vi "Read Value Type Code.vi"(8 "error in (no error)":errorcluster, 11 "NT Scalar in":refnum<class "NT Scalar.lvclass">) -> (0 "error out":errorcluster, 2 "type code":T1, 3 "NT Scalar out":refnum<class "NT Scalar.lvclass">)   [LabVIEW 2020, in "PV Access.lvlib" / "PV Data.lvlib" / "NT Scalar.lvclass"]
uses:
  NT Scalar.lvclass
  NT Scalar.lvclass/NT Scalar.ctl
  1adc147a-9979-490a-b216-bcb4445dfe4b.vi
  Type Code.ctl
  PV Data.lvlib
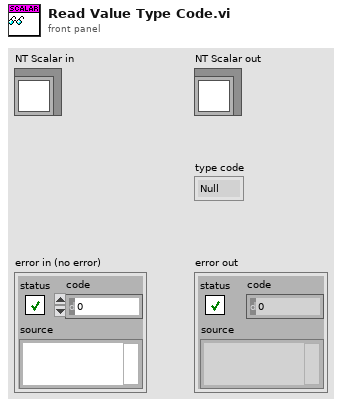
[diagram p1: front panel]
types:
  T1 = typedef "PV Access.lvlib/PV Data.lvlib/Type Code.ctl" = enum8{"Null", "Bool", "BoolA", "Int8", "Int8A", "Int16", "Int16A", "Int32", "Int32A", "Int64", "Int64A", "UInt8", "UInt8A", "UInt16", "UInt16A", "UInt32", "UInt32A", "UInt64", "UInt64A", "Float32", "Float32A", "Float64", "Float64A", "String", "StringA", "Struct", "StructA", "Union", "UnionA", "Any", "AnyA"}
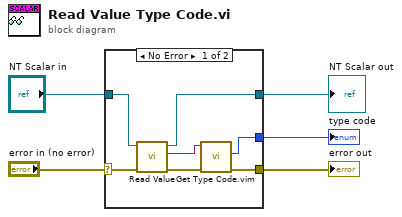
[diagram p0: block diagram]
diagram:
  n1 = case shown="No Error" "error in (no error)" {
    selector: "error in (no error)" -> [w10 w13]
    tunnel: [w7 w13] -> w4
    tunnel: [w11 w14] -> w2
    tunnel: "NT Scalar in" -> [w12 w14]
    tunnel: [w6 _] -> w1
    frame No Error {
      n2 = call-dynamic "Read Value.vi"("error in (no error)"=w10, "NT Scalar in"=w12) -> ("error out"=w8:errorcluster, "value"=w9:variant, "NT Scalar out"=w11:refnum<class "NT Scalar.lvclass">)  [unwired: 7 in]
      n3 = call "Get Type Code.vim"("error in"=w8, "value in"=w9) -> ("error out"=w7:errorcluster, "type code"=w6:T1)  [unwired: 7 in, 1 out]
    }
    frame Error {
    }
  }
  "error out" <- w4
  "NT Scalar out" <- w2
  "type code" <- w1
